vi "RDC-Probe-Calculate_Constants.vi"(11 "Probe Parameters":T1={"lenght [mm]"=50.0, "Core Diameter [mm]"=0.93, "Inner Diameter [mm]"=3.5, "Dieletrisk constant"=2.53}) -> (1 "Vp":dbl, 2 "probe Impedanse":dbl, 3 "Probe Constant K":dbl)   [LabVIEW 2020, in "RDC-Reflection_Data_Computation.lvlib"]
doc: "Computes the propagation velocity Vp, the probe impedance and the probe constant K from the probe parameters (length, core and inner diameter in mm, dielectric constant)."
uses:
  RDC-Reflection_Data_Computation.lvlib
  RDC-Probe_parameters.ctl
panel:
  out "Dieletrisk constant Er":dbl
  out "Inner rad [m] b":dbl
  out "Center rad [m]  a":dbl
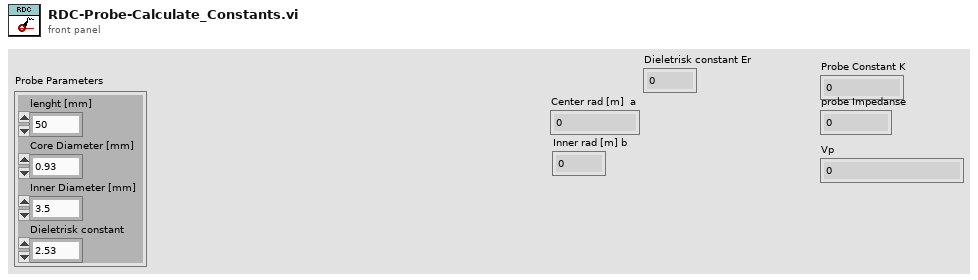
[diagram p1: front panel]
types:
  T1 = typedef "RDC-Reflection_Data_Computation.lvlib/RDC-Probe_parameters.ctl" = cluster{"lenght [mm]":dbl, "Core Diameter [mm]":dbl, "Inner Diameter [mm]":dbl, "Dieletrisk constant":dbl}
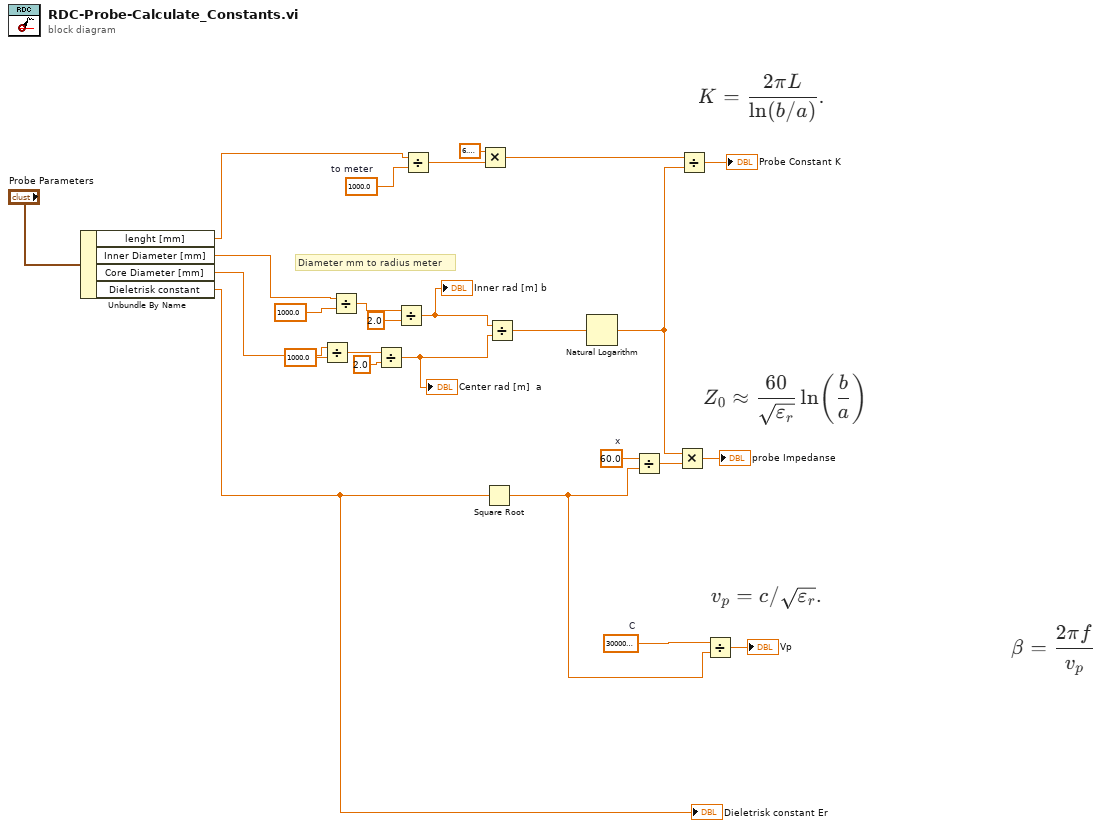
[diagram p0: block diagram]
diagram:
  w10 = 300000000.0  # C
  w14 = 60.0  # x
  w26 = 1000.0  # to meter
  # "Diameter mm to radius meter"
  n1 = Unbundle By Name("Probe Parameters") -> ("lenght [mm]"=w3:dbl, "Inner Diameter [mm]"=w4:dbl, "Core Diameter [mm]"=w5:dbl, "Dieletrisk constant"=w6:dbl)
  "Dieletrisk constant Er" <- w6
  n2 = Divide(x=w5, y=1000.0) -> (x/y=w21:dbl)
  n3 = Divide(x=w4, y=1000.0) -> (x/y=w24:dbl)
  n4 = Divide(x=w21, y=2.0) -> (x/y=w2:dbl)
  "Center rad [m]  a" <- w2
  n5 = Divide(x=w24, y=2.0) -> (x/y=w1:dbl)
  "Inner rad [m] b" <- w1
  n6 = Divide(x=w3, y=w26) -> (x/y=w18:dbl)
  n7 = Multiply(x=6.283185307179586, y=w18) -> (x*y=w16:dbl)
  n8 = Square Root(x=w6) -> (sqrt(x)=w9:dbl)
  n9 = Divide(x=w1, y=w2) -> (x/y=w17:dbl)
  n10 = Natural Logarithm(1:w17) -> (0:w12:dbl)
  n11 = Divide(x=w14, y=w9) -> (x/y=w13:dbl)
  n12 = Multiply(x=w12, y=w13) -> (x*y=→"probe Impedanse":dbl)
  n13 = Divide(x=w16, y=w12) -> (x/y=→"Probe Constant K":dbl)
  n14 = Divide(x=w10, y=w9) -> (x/y=→"Vp":dbl)
